vi "FRC Status Dialog.vi"() -> ()   [LabVIEW 2025]
panel:
  out "progress":u8(slide) scale=0.0..100.0
  out "message":string
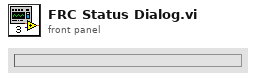
[diagram p1: front panel]
types:
  T1 = cluster{"Quit":bool, "Message":string, "Numeric":u8}
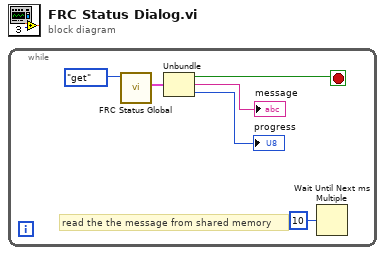
[diagram p0: block diagram]
diagram:
  n1 = while {
    stop <- w5 stop-if-true
    # "read the the message from shared memory"
    n2 = call <resource>:"FRC Status Global.vi"("Mode"=enum16{"get", "set"}."get" ("Switch")) -> ("Data Out"=w2:T1)  [unwired: 9 in, 1 out]
    n3 = Unbundle(w2) -> ("Quit"=w5:bool, "Message"=→"message":string, "Numeric"=→"progress":u8)
    n4 = Wait Until Next ms Multiple(millisecond multiple=u32 10) -> ()  [unwired: 1 out]
  }
